vi "Get Image From FrontPanel.vi"(6 "Bounds":T1, 8 "error in (no error)":errorcluster, 11 "vi reference":refnum<vi>) -> (0 "error out":errorcluster, 1 "image size":T2, 2 "image":picture, 3 "reference out":refnum<vi>)   [LabVIEW 2019, in "Language Editor.lvlib"]
doc: "- - -\nCopyright (c) 2026, Merecs Engineering GmbH"
uses:
  Language Editor.lvlib
  <vilib>/Utility/miscctls.llb/LVBoundsTypeDef.ctl
  <vilib>/Utility/miscctls.llb/LVPointTypeDef.ctl
panel:
  # "Connector Pane"
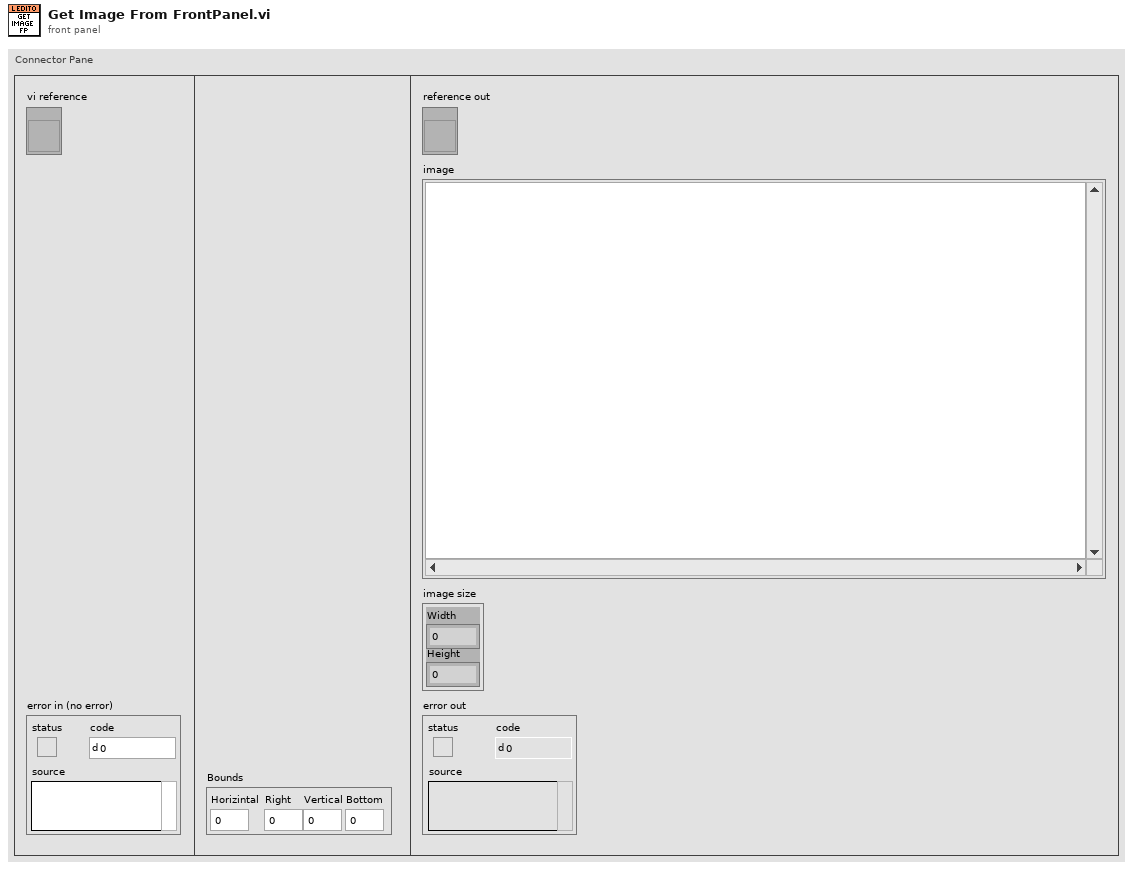
[diagram p1: front panel]
types:
  T1 = cluster{"Horizintal":i32, "Right":i32, "Vertical":i32, "Bottom":i32}
  T2 = typedef "LVBoundsTypeDef.ctl" = cluster{"Width":u32, "Height":u32}
  T3 = typedef "LVPointTypeDef.ctl" = cluster{"Horizontal":i16, "Vertical":i16}
  T4 = typedef "LVRectTypeDef.ctl" = cluster{"Left":i16, "Top":i16, "Right":i16, "Bottom":i16}
  T5 = typedef "imagedata.ctl" = cluster{"image type":i32, "image depth":i32, "image":u8[], "mask":u8[], "colors":u32[], "Rectangle":cluster{"left":i16, "top":i16, "right":i16, "bottom":i16}}
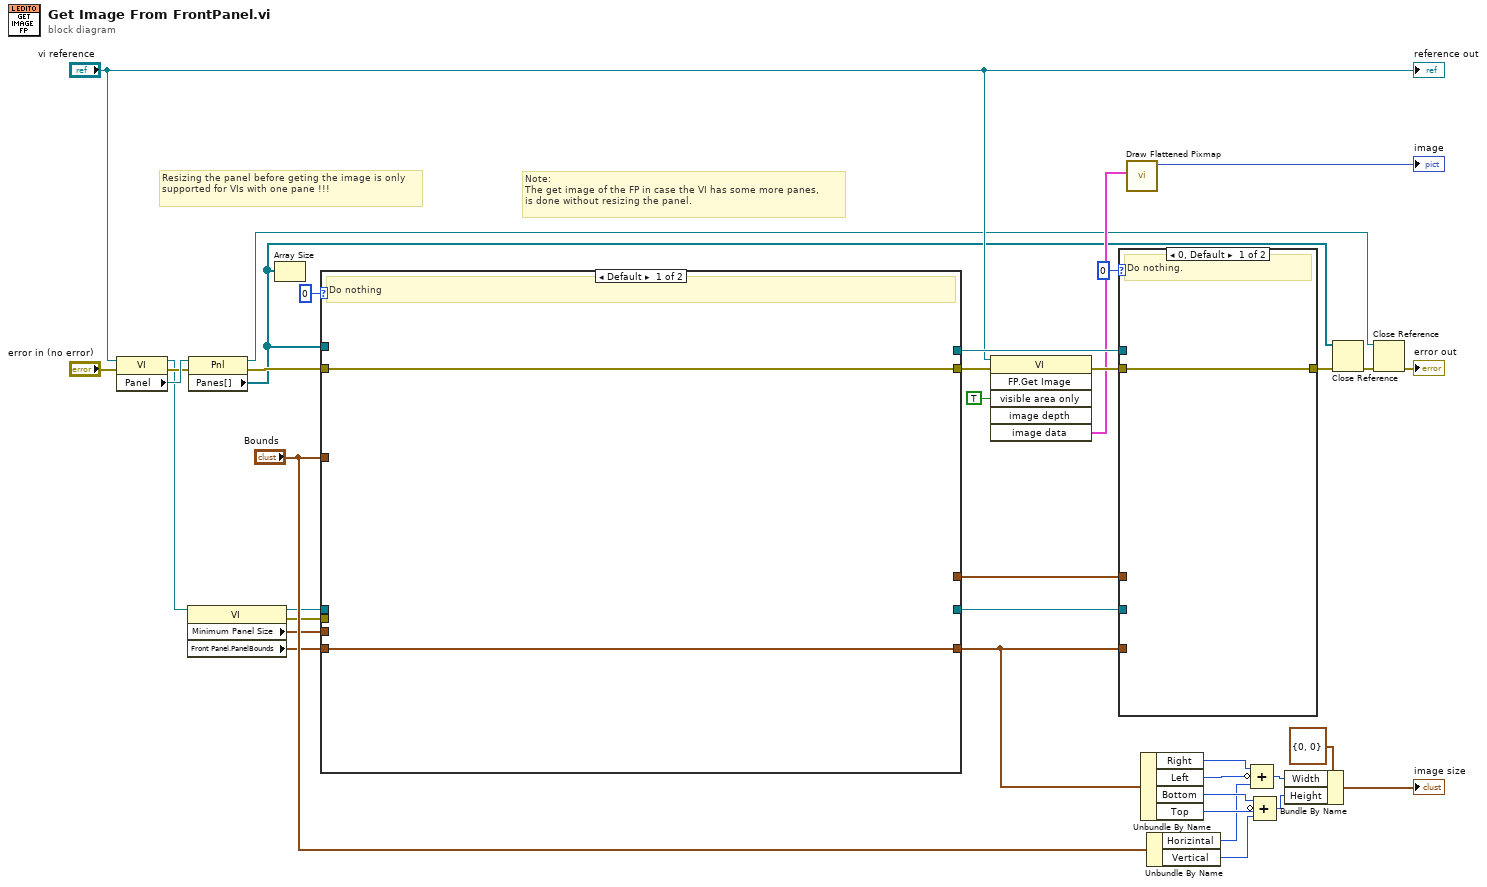
[diagram p0: block diagram]
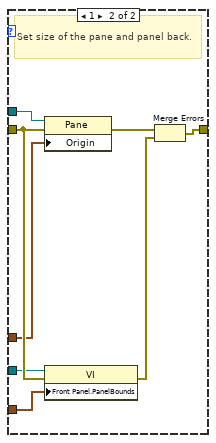
[diagram p2: hidden frame]
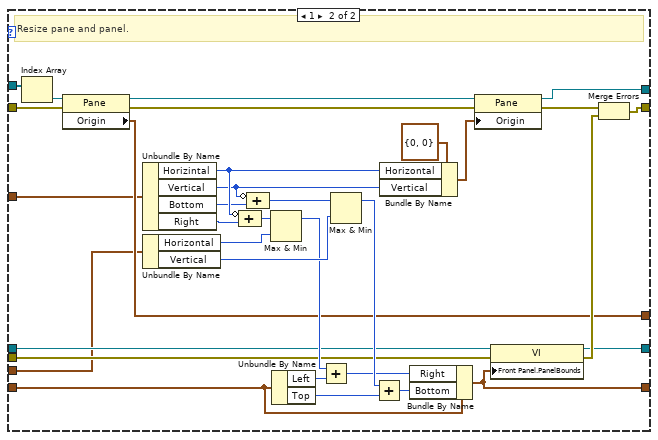
[diagram p3: hidden frame]
diagram:
  # "Note:\nThe get image of the FP in case the VI has some more panes,\nis done without resizing the panel."
  # "Resizing the panel before geting the image is only supported for VIs with one pane !!!"
  n1 = property class="VI"(reference="vi reference", error in="error in (no error)") -> (reference out=w5:refnum<vi>, error out=w33:errorcluster, "Panel"=w35:refnum<vi>)
  n2 = property class="VI"(reference=w5) -> (reference out=w8:refnum<vi>, error out=w7:errorcluster, "Minimum Panel Size"=w4:T3, "Front Panel.PanelBounds"=w6:T4)  [unwired: 1 in]
  n3 = property class="Pnl"(reference=w35, error in=w33) -> (reference out=w12:refnum<vi>, error out=w32:errorcluster, "Panes[]"=w13:refnum<vi>[])
  n4 = Array Size(array=w13) -> ()  [unwired: 1 out]
  n5 = case shown="Default" 0 {
    tunnel: [_ w66] -> w34
    tunnel: [_ w63] -> w28
    tunnel: w13 -> [_ w62]
    tunnel: w32 -> [w39 w68]
    tunnel: [w39 w61] -> w31
    tunnel: [_ w59] -> w30
    tunnel: "Bounds" -> [_ w52]
    tunnel: w8 -> [_ w44]
    tunnel: w7 -> [_ w43]
    tunnel: w6 -> [w38 w41]
    tunnel: w4 -> [_ w42]
    tunnel: [w38 w40] -> w3
    frame Default {
      # "Do nothing"
    }
    frame 1 {
      # "Resize pane and panel."
      n6 = Index Array(array=w62) -> (element=w64:refnum<vi>)  [unwired: 1 in]
      n7 = property class="Pane"(reference=w64, error in=w68) -> (reference out=w65:refnum<vi>, error out=w56:errorcluster, "Origin"=w59:T3)
      n8 = Unbundle By Name(w52) -> ("Horizintal"=w55:i32, "Vertical"=w53:i32, "Bottom"=w54:i32, "Right"=w51:i32)
      n9 = Unbundle By Name(w42) -> ("Horizontal"=w70:i16, "Vertical"=w72:i16)
      n10 = Compound Arithmetic op=ADD(invert w55, w51) -> (w47:i32)
      n11 = Compound Arithmetic op=ADD(invert w53, w54) -> (w50:i32)
      n12 = Max & Min(x=w47, y=w70) -> (max(x,y)=w69:i32)  [unwired: 1 out]
      n13 = Unbundle By Name(w41) -> ("Left"=w46:i16, "Top"=w49:i16)
      n14 = Add(x=w69, y=w46) -> (x+y=w45:i32)
      n15 = Max & Min(x=w50, y=w72) -> (max(x,y)=w71:i32)  [unwired: 1 out]
      n16 = Add(x=w71, y=w49) -> (x+y=w48:i32)
      n17 = Bundle By Name(cluster=T3 {"Horizontal"=0, "Vertical"=0} ("OriginOffset"), "Horizontal"=w55, "Vertical"=w53) -> (w57:T3)
      n18 = Bundle By Name(cluster=w41, "Right"=w45, "Bottom"=w48) -> (w40:T4)
      n19 = property class="Pane"(reference=w65, error in=w56, "Origin"=w57) -> (reference out=w63:refnum<vi>, error out=w60:errorcluster)
      n20 = property class="VI"(reference=w44, error in=w43, "Front Panel.PanelBounds"=w40) -> (reference out=w66:refnum<vi>, error out=w67:errorcluster)
      n21 = Merge Errors(w60, w67) -> (w61:errorcluster)
    }
  }
  n22 = invoke class="VI" method="FP.Get Image"(reference="vi reference", error in=w31, "visible area only"=TRUE ("Visible Area Only")) -> (error out=w29:errorcluster, "image data"=w18:T5)  [unwired: 3 in, 4 out]
  n23 = case shown="0, Default" 0 {
    tunnel: w34 -> [_ w80]
    tunnel: w3 -> [_ w79]
    tunnel: w28 -> [_ w78]
    tunnel: w30 -> [_ w77]
    tunnel: w29 -> [w73 w81]
    tunnel: [w73 w74] -> w17
    frame 0, Default {
      # "Do nothing."
    }
    frame 1 {
      # "Set size of the pane and panel back."
      n24 = property class="Pane"(reference=w78, error in=w81, "Origin"=w77) -> (error out=w76:errorcluster)  [unwired: 1 out]
      n25 = property class="VI"(reference=w80, error in=w81, "Front Panel.PanelBounds"=w79) -> (error out=w75:errorcluster)  [unwired: 1 out]
      n26 = Merge Errors(w76, w75) -> (w74:errorcluster)
    }
  }
  n27 = call <vilib>:"Draw Flattened Pixmap.vi"("image data"=w18) -> ("new picture"=→"image":picture)  [unwired: 8 in]
  n28 = Unbundle By Name(w3) -> ("Right"=w20:i16, "Left"=w21:i16, "Bottom"=w22:i16, "Top"=w23:i16)
  n29 = Unbundle By Name("Bounds") -> ("Horizintal"=w10:i32, "Vertical"=w9:i32)
  n30 = Compound Arithmetic op=ADD(w20, invert w21, w10) -> (w25:i32)
  n31 = Compound Arithmetic op=ADD(w22, invert w23, w9) -> (w26:i32)
  n32 = Bundle By Name(cluster=T2 {"Width"=0, "Height"=0} ("Draw Area Size"), "Width"=w25, "Height"=w26) -> (→"image size":T2)
  n33 = Close Reference(reference=w13, error in (no error)=w17) -> (error out=w15:errorcluster)
  n34 = Close Reference(reference=w12, error in (no error)=w15) -> (error out=→"error out":errorcluster)
  "reference out" <- "vi reference"
